vi "GOOP_LVClass_Provider_OnPopupMenu.vi"(11 "objects":T1[](array[typedef])) -> ()   [LabVIEW 2020]
uses:
  <resource>/Framework/Providers/API/ItemRef.ctl
  <resource>/Framework/Providers/API/mxLvMenuItem.ctl
panel:
  out "error out":errorcluster
  in  "error in":errorcluster
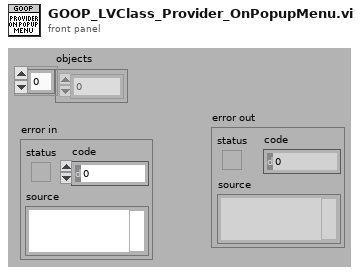
[diagram p1: front panel]
types:
  T1 = typedef "ItemRef.ctl" = u64
  T2 = typedef "mxLvMenuItem.ctl" = cluster{"Menu Name":string, "Description":string, "Icon File Name":path, "Menu Tag":string, "Enabled":bool, "Checked":bool, "Separator":bool, "Batchable":bool, "Weight":i32, "Batch Mode (Ignored if Not Batchable)":enum32{"Show If All Items Support Command", "Show If Any Items Support Command"}, "Menu Location":enum32{"<None>", "Project", "Project / Build Specifications", "Tools", "Tools / Source Control", "Tools / Real-Time Module", "Help"}, "Exclude From Getting Started Window Menu":bool}
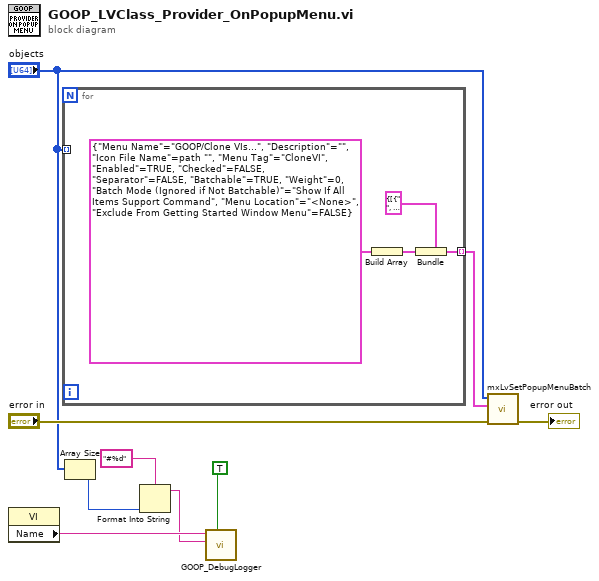
[diagram p0: block diagram]
diagram:
  n1 = property class="VI"() -> ("Name"=w7:string)  [unwired: 2 in, 2 out]
  n2 = for {
    tunnel: [w12] -> w6 mode=indexing
    tunnel: "objects" -> [_] mode=indexing
    n3 = Build Array(T2 {"Menu Name"="GOOP/Clone VIs...", "Description"="", "Icon File Name"=path "", "Menu Tag"="CloneVI", "Enabled"=TRUE, "Checked"=FALSE, "Separator"=FALSE, "Batchable"=TRUE, "Weight"=0, "Batch Mode (Ignored if Not Batchable)"=enum."Show If All Items Support Command", "Menu Location"=enum."<None>", "Exclude From Getting Started Window Menu"=FALSE} ("Menu Item")) -> (w13:T2[])
    n4 = Bundle(cluster=cluster{"Popup Menu Items":T2[]} {"Popup Menu Items"=[{"Menu Name"="", "Description"="", "Icon File Name"=path "", "Menu Tag"="", "Enabled"=TRUE, "Checked"=FALSE, "Separator"=FALSE, "Batchable"=TRUE, "Weight"=0, "Batch Mode (Ignored if Not Batchable)"=enum."Show If Any Items Support Command", "Menu Location"=enum."<None>", "Exclude From Getting Started Window Menu"=FALSE}]}, "Popup Menu Items"=w13) -> (w12:cluster{"Popup Menu Items":T2[]})
  }
  n5 = Array Size(array="objects") -> (size(s)=w2:i32)
  n6 = Format Into String(format string="#%d", w2) -> (resulting string=w1:string)  [unwired: 2 in, 1 out]
  n7 = call <resource>:"GOOP_DebugLogger.vi"("ActivateDebugging"=TRUE, "Data"=w1, "State"=w7) -> ()  [unwired: 6 in, 3 out]
  n8 = call <resource>:"mxLvSetPopupMenuBatch.vi"("error in"="error in", "Menu Items"=w6, "Items"="objects") -> ("error out"=→"error out":errorcluster)  [unwired: 7 in, 1 out]
